vi "SDO_TRAJECTORY_EXECUTE_ABS.vi"(6 "EnableClosedLoop":bool=TRUE, 8 "Init":bool, 11 "End Pose ENG":T1={"TRANSLATION"={"X"=0.0, "Y"=0.0}, "ROTATION"={"VALUE"=0.0, "COS"=1.0, "SIN"=0.0}} {"ROTATION"."SIN" format="%13.4f"; "ROTATION"."COS" format="%13.4f"; "ROTATION"."VALUE" format="%13.4f"; "TRANSLATION"."Y" format="%14.3f"; "TRANSLATION"."X" format="%14.3f"}) -> (0 "AtReference":bool, 3 "Chassis Velocity Target":T4 {"vOmega" format="%10.3f"; "vY" format="%10.3f"; "vX" format="%10.3f"})   [LabVIEW 2019]
uses:
  <vilib>/Rock Robotics/WPI/ThirdParty/JAS_Junk/TrajLib/TypeDef/CHASSIS_SPEEDS.ctl
  <vilib>/Rock Robotics/WPI/ThirdParty/JAS_Junk/TrajLib/VI/Util_GetTime_U32.vi
  <vilib>/Rock Robotics/WPI/ThirdParty/JAS_Junk/TrajLib/ProfiledPIDController_NewPeriod.vi
  <vilib>/Rock Robotics/WPI/ThirdParty/JAS_Junk/TrajLib/ProfiledPIDController_SetIntegratorRange.vi
  <vilib>/Rock Robotics/WPI/ThirdParty/JAS_Junk/TrajLib/ProfiledPIDController_DisableContInput.vi
  <vilib>/Rock Robotics/WPI/ThirdParty/JAS_Junk/TrajLib/ProfiledPIDController_EnableContInput.vi
  <vilib>/Rock Robotics/WPI/ThirdParty/JAS_Junk/TrajLib/TrapProfConstraint_New.vi
  <vilib>/Rock Robotics/WPI/ThirdParty/JAS_Junk/TrajLib/Rotation2d_CreateAngle.vi
  <vilib>/Rock Robotics/WPI/ThirdParty/JAS_Junk/TrajLib/Translation2d_Create.vi
  <vilib>/Rock Robotics/WPI/ThirdParty/JAS_Junk/TrajLib/HolDrvCtrl_New.vi
  <vilib>/Rock Robotics/WPI/ThirdParty/JAS_Junk/TrajLib/HolDrvCtrl_PackPID.vi
  <vilib>/Rock Robotics/WPI/ThirdParty/JAS_Junk/TrajLib/HolDrvCtrl_SetTolerance.vi
  <vilib>/Rock Robotics/WPI/ThirdParty/JAS_Junk/TrajLib/HolDrvCtrl_SetEnabled.vi
  <vilib>/Rock Robotics/WPI/ThirdParty/JAS_Junk/TrajLib/HolDrvCtrl_Calculate_Trajectory.vi
  <vilib>/Rock Robotics/WPI/ThirdParty/JAS_Junk/TrajLib/HolDrvCtrl_AtReference.vi
  <vilib>/Rock Robotics/WPI/ThirdParty/JAS_Junk/TrajLib/TrapProfState_New.vi
  <vilib>/Rock Robotics/WPI/ThirdParty/JAS_Junk/TrajLib/PIDController_NewPeriod.vi
  <vilib>/Rock Robotics/SystemInterfaces/NetworkCommunication/NetComm_UsageReport_report.vi
  <vilib>/Rock Robotics/WPI/ThirdParty/JAS_Junk/TrajLib/PIDController_SetIntegratorRange.vi
  <vilib>/Rock Robotics/WPI/ThirdParty/JAS_Junk/TrajLib/PIDController_DisableContinousInput.vi
  <vilib>/Rock Robotics/WPI/ThirdParty/JAS_Junk/TrajLib/PIDController_EnableContinousInput.vi
  <vilib>/Rock Robotics/WPI/ThirdParty/JAS_Junk/TrajLib/Conv_Deg_Radians.vi
  <vilib>/Rock Robotics/WPI/ThirdParty/JAS_Junk/TrajLib/PIDController_Reset.vi
  <vilib>/Rock Robotics/WPI/ThirdParty/JAS_Junk/TrajLib/HolDrvCtrl_Calculate.vi
  <vilib>/Rock Robotics/WPI/ThirdParty/JAS_Junk/TrajLib/Rotation2d_GetRadians.vi
  <vilib>/Rock Robotics/WPI/ThirdParty/JAS_Junk/TrajLib/Rotation2d_GetAngleCosSin.vi
  <vilib>/Rock Robotics/WPI/ThirdParty/JAS_Junk/TrajLib/Pose2d_RelativeTo.vi
  <vilib>/Rock Robotics/WPI/ThirdParty/JAS_Junk/TrajLib/Pose2d_getRotation.vi
  <vilib>/Rock Robotics/WPI/ThirdParty/JAS_Junk/TrajLib/Rotation2d_Minus.vi
  <vilib>/Rock Robotics/WPI/ThirdParty/JAS_Junk/TrajLib/ProfiledPIDController_Calculate_Meas_Goal.vi
  <vilib>/Rock Robotics/WPI/ThirdParty/JAS_Junk/TrajLib/ChassisSpeeds_FromFieldRelativeSpeeds.vi
  <vilib>/Rock Robotics/WPI/ThirdParty/JAS_Junk/TrajLib/PIDController_Calculate_SP_PV.vi
  <vilib>/Rock Robotics/WPI/ThirdParty/JAS_Junk/TrajLib/ProfiledPIDController_Reset_PosOnly.vi
  <vilib>/Rock Robotics/WPI/ThirdParty/JAS_Junk/TrajLib/Rotation2d_Plus.vi
  <vilib>/Rock Robotics/WPI/ThirdParty/JAS_Junk/TrajLib/Transform2d_Create_PosePose.vi
  <vilib>/Rock Robotics/WPI/ThirdParty/JAS_Junk/TrajLib/Pose2d_New_TRRO.vi
  <vilib>/Rock Robotics/WPI/ThirdParty/JAS_Junk/TrajLib/Rotation2d_UnaryMinus.vi
  <vilib>/Rock Robotics/WPI/ThirdParty/JAS_Junk/TrajLib/Rotation2d_RotateBy.vi
  <vilib>/Rock Robotics/WPI/ThirdParty/JAS_Junk/TrajLib/ProfiledPIDController_SetGoal_PosOnly.vi
  <vilib>/Rock Robotics/WPI/ThirdParty/JAS_Junk/TrajLib/ProfiledPIDController_Calculate_Meas.vi
  <vilib>/Rock Robotics/WPI/ThirdParty/JAS_Junk/TrajLib/Rotation2d_GetCos.vi
  <vilib>/Rock Robotics/WPI/ThirdParty/JAS_Junk/TrajLib/Rotation2d_GetSin.vi
  <vilib>/Rock Robotics/WPI/ThirdParty/JAS_Junk/TrajLib/PIDController_SetSetpoint.vi
  <vilib>/Rock Robotics/WPI/ThirdParty/JAS_Junk/TrajLib/PIDController_Calculate_PV.vi
  <vilib>/Rock Robotics/WPI/ThirdParty/JAS_Junk/TrajLib/ProfiledPIDController_Reset.vi
  <vilib>/Rock Robotics/WPI/ThirdParty/JAS_Junk/TrajLib/Translation2d_RotateBy.vi
  <vilib>/Rock Robotics/WPI/ThirdParty/JAS_Junk/TrajLib/Translation2d_Minus.vi
  <vilib>/Rock Robotics/WPI/ThirdParty/JAS_Junk/TrajLib/Rotation2d_CreateXY.vi
  <vilib>/Rock Robotics/WPI/ThirdParty/JAS_Junk/TrajLib/ProfiledPIDController_SetGoal.vi
  <vilib>/Rock Robotics/WPI/ThirdParty/JAS_Junk/TrajLib/TrapProfile_New.vi
  <vilib>/Rock Robotics/WPI/ThirdParty/JAS_Junk/TrajLib/ProfiledPIDController_GetPeriod.vi
  <vilib>/Rock Robotics/WPI/ThirdParty/JAS_Junk/TrajLib/TrapProfile_Calculate.vi
  <vilib>/Rock Robotics/WPI/ThirdParty/JAS_Junk/TrajLib/ControllerUtil_GetModulusError.vi
  <vilib>/Rock Robotics/WPI/ThirdParty/JAS_Junk/TrajLib/Util_CalcDist.vi
  <vilib>/Rock Robotics/WPI/ThirdParty/JAS_Junk/TrajLib/TrapProfile_ShouldFlipAcceleration.vi
  <vilib>/Rock Robotics/WPI/ThirdParty/JAS_Junk/TrajLib/TrapProfile_Direct.vi
  <vilib>/Rock Robotics/WPI/ThirdParty/JAS_Junk/TrajLib/PIDController_GetPeriod.vi
  Swerve_Drive_System/SDO_DRIVE_GLOBALS.vi
  <vilib>/Rock Robotics/WPI/ThirdParty/JAS_Junk/TrajLib/VI/Util_GetTime_U64.vi
  SDO_TRAJECTORY_GLOBALS.vi
  <vilib>/Rock Robotics/WPI/ThirdParty/JAS_Junk/TrajLib/Globals/Util_LibraryGlobals.vi
  <vilib>/Rock Robotics/WPI/ThirdParty/JAS_Junk/TrajLib/Trajectory_Library.lvlib
  <vilib>/Rock Robotics/WPI/ThirdParty/JAS_Junk/TrajLib/TypeDef/TRANSLATION2D.ctl
  <vilib>/Rock Robotics/WPI/ThirdParty/JAS_Junk/TrajLib/TypeDef/ROTATION2D.ctl
  <vilib>/Rock Robotics/WPI/ThirdParty/JAS_Junk/TrajLib/TypeDef/POSE2D.ctl
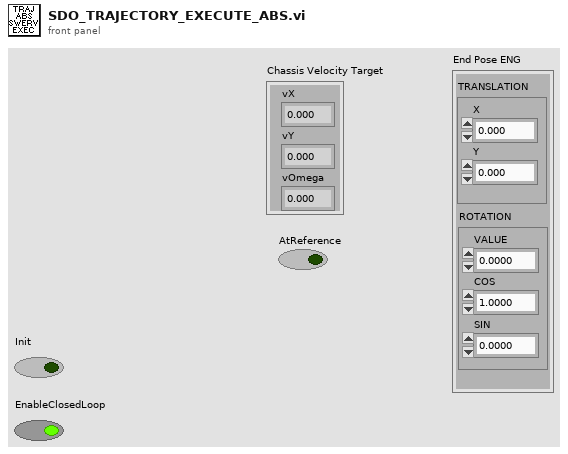
[diagram p1: front panel]
types:
  T1 = typedef "Trajectory_Library.lvlib/POSE2D.ctl" = cluster{"TRANSLATION":T2, "ROTATION":T3}
  T2 = typedef "Trajectory_Library.lvlib/TRANSLATION2D.ctl" = cluster{"X":dbl, "Y":dbl}
  T3 = typedef "Trajectory_Library.lvlib/ROTATION2D.ctl" = cluster{"VALUE":dbl, "COS":dbl, "SIN":dbl}
  T4 = typedef "Trajectory_Library.lvlib/CHASSIS_SPEEDS.ctl" = cluster{"vX":dbl, "vY":dbl, "vOmega":dbl}
  T5 = typedef "Trajectory_Library.lvlib/SWERVE_DRIVE_KINEMATICS.ctl" = cluster{"NumModules":i32, "InverseKinematics":T6, "ForwardKinematics":T6, "Modules":T2[], "PrevCoR":T2, "SavedModuleStates":T7[]}
  T6 = typedef "NI_Matrix.lvlib/RealMatrix.ctl" = dbl[][]
  T7 = typedef "Trajectory_Library.lvlib/SWERVE_DRIVE_MODULE_STATE.ctl" = cluster{"Speed":dbl, "Angle":T3}
  T8 = typedef "Trajectory_Library.lvlib/TRAJECTORY.ctl" = cluster{"TotalTImeSecs":dbl, "States":T9[]}
  T9 = typedef "Trajectory_Library.lvlib/TRAJ_STATE.ctl" = cluster{"TimeSeconds":dbl, "Velocity":dbl, "Acceleration":dbl, "POSE":T1, "Curvature":dbl}
  T10 = typedef "Trajectory_Library.lvlib/PID_TUNING.ctl" = cluster{"Kp":dbl, "Ki":dbl, "Kd":dbl, "MaximumIntegral":dbl, "MinimumIntegral":dbl}
  T11 = typedef "Trajectory_Library.lvlib/PROFILED_PID_CONTROLLER.ctl" = cluster{"Controller":T12, "Goal":T13, "Setpoint":T13, "Constraint":T14}
  T12 = typedef "Trajectory_Library.lvlib/PID_CONTROLLER.ctl" = cluster{"Kp":dbl, "Ki":dbl, "Kd":dbl, "Period":dbl, "Max_Integral":dbl, "Min_Integral":dbl, "Max_Input":dbl, "Min_Input":dbl, "Continuous":bool, "PositionError":dbl, "VelocityError":dbl, "PrevError":dbl, "TotalError":dbl, "PositionTolerance":dbl, "VelocityTolerance":dbl, "SetPoint":dbl, "Kf":dbl, "Prev_Deriv":dbl, "Prev_Deriv 2":dbl, "DerivativeFilter":bool, "Min_Output":dbl, "Max_Output":dbl, "Prev_F_P":dbl, "Prev_F_P_2":dbl, "AntiWindupActive":bool, "Measurement":dbl}
  T13 = typedef "Trajectory_Library.lvlib/TRAPEZOID_PROFILE_STATE.ctl" = cluster{"Position":dbl, "Velocity":dbl}
  T14 = typedef "Trajectory_Library.lvlib/TRAPEZOID_PROFILE_CONSTRAINT.ctl" = cluster{"MaxVelocity":dbl, "MaxAcceleration":dbl}
  T15 = typedef "Trajectory_Library.lvlib/HOLONOMIC_PACK_TUNING.ctl" = cluster{"X PID Tuning":T10, "Y PID Tuning":T10, "thetaProfiledPID_CTRL":T11}
  T16 = typedef "Trajectory_Library.lvlib/HOLONOMIC_DRV_CTRL.ctl" = cluster{"poseTolerance":T1, "poseError":T1, "Enabled":bool, "PID_xCtrl":T12, "PID_yCtrl":T12, "PROF_PID_thetaCtrl":T11, "RotationError":T3, "FirstRun":bool}
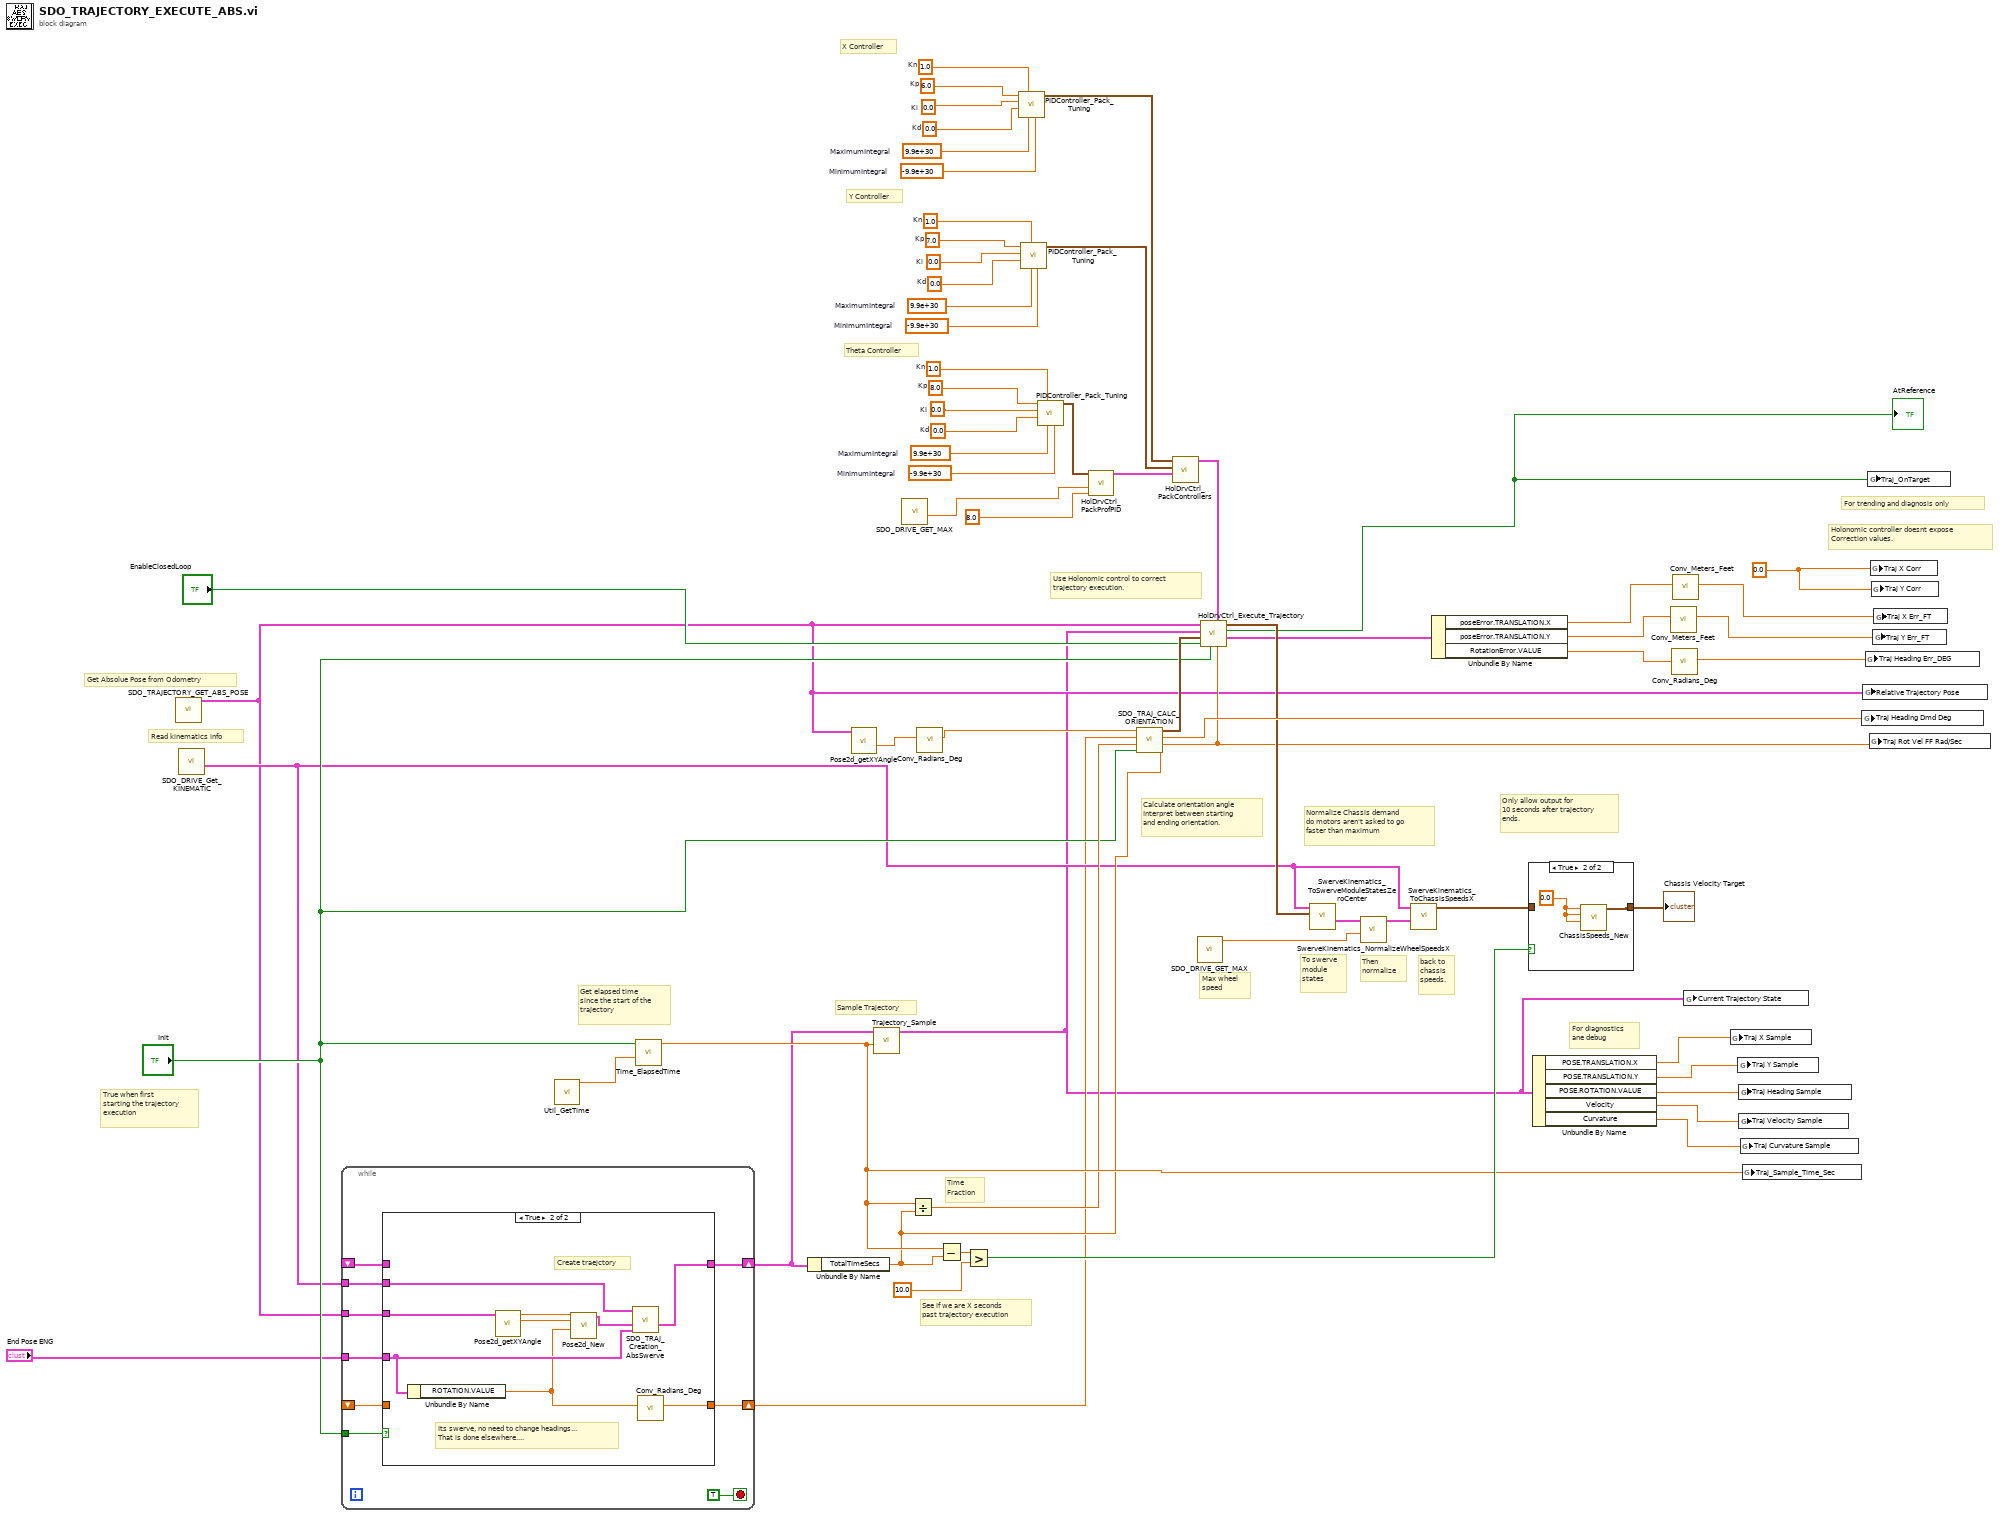
[diagram p0: block diagram]
diagram:
  w23 = 1.0  # Kn
  w26 = 8.0  # Kp
  w35 = 0.0  # Ki
  w36 = 0.0  # Kd
  w37 = 9.9e+30  # MaximumIntegral
  w38 = -9.9e+30  # MinimumIntegral
  w21 = 1.0  # Kn
  w24 = 6.0  # Kp
  w27 = 0.0  # Ki
  w28 = 0.0  # Kd
  w29 = 9.9e+30  # MaximumIntegral
  w30 = -9.9e+30  # MinimumIntegral
  w22 = 1.0  # Kn
  w25 = 7.0  # Kp
  w31 = 0.0  # Ki
  w32 = 0.0  # Kd
  w33 = 9.9e+30  # MaximumIntegral
  w34 = -9.9e+30  # MinimumIntegral
  w51 = 0.0 ("Y Corr")
  # "Theta Controller"
  # "Y Controller"
  # "X Controller"
  # "Time\nFraction"
  # "Calculate orientation angle\nInterpret between starting\nand ending orientation."
  # "Max wheel\nspeed"
  # "True when first\nstarting the trajectory\nexecution"
  # "Get elapsed time\nsince the start of the\ntrajectory"
  # "Holonomic controller doesnt expose\nCorrection values."
  # "Normalize Chassis demand\ndo motors aren't asked to go\nfaster than maximum"
  # "Use Holonomic control to correct\ntrajectory execution."
  # "For trending and diagnosis only"
  # "For diagnostics\nane debug"
  # "Get Absolue Pose from Odometry"
  # "back to\nchassis\nspeeds."
  # "Then\nnormalize"
  # "To swerve\nmodule\nstates"
  # "Read kinematics info"
  # "Sample Trajectory"
  # "See if we are X seconds \npast trajectory execution"
  # "Only allow output for\n10 seconds after trajectory\nends."
  n1 = call "SDO_TRAJECTORY_GET_ABS_POSE.vi"() -> ("Absolute Odometry Pose"=w6:T1)  [unwired: 11 in]
  n2 = call "SDO_DRIVE_Get_KINEMATIC.vi"() -> ("out SWERVE_DRIVE_KINEMATICS"=w8:T5)  [unwired: 11 in]
  n3 = while {
    tunnel: "Init" -> [w73]
    tunnel: w8 -> [w72]
    tunnel: w6 -> [w71]
    shift-right: [w70] -> w7
    shift-left: _ -> [w69]
    shift-right: [w68] -> w3
    shift-left: _ -> [w67]
    tunnel: "End Pose ENG" -> [w66]
    stop <- TRUE stop-if-true
    n4 = case shown="True" w73 {
      tunnel: w72 -> [_ w85]
      tunnel: w71 -> [_ w83]
      tunnel: [w76 w84] -> w70
      tunnel: w69 -> [w76 _]
      tunnel: [w75 w78] -> w68
      tunnel: w67 -> [w75 _]
      tunnel: w66 -> [_ w79]
      frame False {
      }
      frame True {
        # "Its swerve, no need to change headings...\nThat is done elsewhere...."
        # "Create traejctory"
        n5 = Unbundle By Name(w79) -> ("ROTATION.VALUE"=w77:dbl)
        n6 = call <vilib>:"Pose2d_getXYAngle.vi"("in POSE"=w83) -> ("Y"=w81:dbl, "X"=w82:dbl)  [unwired: 8 in, 1 out]
        n7 = call <vilib>:"Pose2d_New.vi"("Heading"=w77, "Y"=w81, "X"=w82) -> ("out POSe"=w80:T1)  [unwired: 8 in]
        n8 = call "SDO_TRAJ_Creation_AbsSwerve.vi"("End Pose  ENG"=w79, "Current Pose SI"=w80, "SWERVE_DRIVE_KINEMATICS"=w85) -> ("Absolute Trajectory"=w84:T8)  [unwired: 6 in, 2 out]
        n9 = call <vilib>:"Conv_Radians_Deg.vi"("Radians"=w77) -> ("Degrees"=w78:dbl)  [unwired: 10 in]
      }
    }
  }
  n10 = call <vilib>:"Util_GetTime.vi"() -> ("FPGA_Time_Seconds"=w57:dbl)  [unwired: 9 in, 2 out]
  n11 = call <vilib>:"Time_ElapsedTime.vi"("PassthroughTime_SEC"=w57, "Reset"="Init") -> ("Elapsed Time Sec"=w49:dbl)  [unwired: 9 in]
  n12 = Unbundle By Name(w7) -> ("TotalTImeSecs"=w12:dbl)
  n13 = call <vilib>:"Pose2d_getXYAngle.vi"("in POSE"=w6) -> ("Angle"=w5:dbl)  [unwired: 8 in, 2 out]
  n14 = call <vilib>:"Trajectory_Sample.vi"("Time"=w49, "InputTRAJECTORY"=w7) -> ("OutputTRAJ_STATE"=w2:T9)  [unwired: 9 in]
  n15 = call "SDO_DRIVE_GET_MAX.vi"() -> ("Max Rotational Vel (Rad/Sec)"=w11:dbl)  [unwired: 10 in, 1 out]
  n16 = Divide(x=w49, y=w12) -> (x/y=w48:dbl)
  n17 = call <vilib>:"Conv_Radians_Deg.vi"("Radians"=w5) -> ("Degrees"=w4:dbl)  [unwired: 10 in]
  n18 = Subtract(x=w49, y=w12) -> (x-y=w65:dbl)
  n19 = Greater?(x=w65, y=10.0) -> (0:w63:bool)
  n20 = call <vilib>:"PIDController_Pack_Tuning.vi"("MinimumIntegral"=w30, "MaximumIntegral"=w29, "Kn"=w21, "Kd"=w28, "Ki"=w27, "Kp"=w24) -> ("PID Tuning"=w39:T10)  [unwired: 5 in]
  n21 = call <vilib>:"PIDController_Pack_Tuning.vi"("MinimumIntegral"=w34, "MaximumIntegral"=w33, "Kn"=w22, "Kd"=w32, "Ki"=w31, "Kp"=w25) -> ("PID Tuning"=w40:T10)  [unwired: 5 in]
  n22 = call <vilib>:"PIDController_Pack_Tuning.vi"("MinimumIntegral"=w38, "MaximumIntegral"=w37, "Kn"=w23, "Kd"=w36, "Ki"=w35, "Kp"=w26) -> ("PID Tuning"=w20:T10)  [unwired: 5 in]
  n23 = call <vilib>:"HolDrvCtrl_PackProfPID.vi"("Max Accel"=8.0, "Max Speed"=w11, "Theta PID Tuning"=w20) -> ("Theta PID CONTROLLER"=w41:T11)  [unwired: 8 in]
  n24 = call "SDO_TRAJ_CALC_ORIENTATION.vi"("Total Trajectory Time"=w12, "Init"="Init", "Time Fraction"=w48, "End Orientation Demand DEG"=w3, "Starting Orientation  DEG"=w4) -> ("Rotational Velocity"=w15:dbl, "Orientation Demand Deg"=w50:dbl, "Orientation Demand"=w19:T3)  [unwired: 4 in]
  n25 = call <vilib>:"HolDrvCtrl_PackControllers.vi"("thetaProfiledPID_CTRL"=w41, "Y PID Tuning"=w40, "X PID Tuning"=w39) -> ("HOLONOMIC_CTRL_PACK_TUNING"=w42:T15)  [unwired: 8 in]
  n26 = call "SDO_DRIVE_GET_MAX.vi"() -> ("Max Wheel Vel (Meter/Sec)"=w59:dbl)  [unwired: 10 in, 1 out]
  n27 = call <vilib>:"HolDrvCtrl_Execute_Trajectory.vi"("Rotational Velocity Feedforward \nRad/Sec"=w15, "HOLONOMIC_CTRL_PACK_TUNING"=w42, "Reset"="Init", "Enable"="EnableClosedLoop", "angleRef"=w19, "desiredTrajState"=w2, "currentPose"=w6) -> ("outHOLONOMIC_DRV_CTRL"=w16:T16, "AtReference"=w17:bool, "calcChassisSpeed"=w18:T4)  [unwired: 2 in]
  "AtReference" <- w17
  n28 = call <vilib>:"SwerveKinematics_ToSwerveModuleStatesZeroCenter.vi"("ChassisSpeeds"=w18, "in SWERVE_DRIVE_KINEMATICS"=w8) -> ("ModuleStates"=w62:T7[])  [unwired: 8 in, 1 out]
  n29 = call <vilib>:"SwerveKinematics_NormalizeWheelSpeedsX.vi"("AttainableMaxSpeed"=w59, "in WheelStates"=w62) -> ("out WheelStates"=w61:T7[])  [unwired: 9 in]
  n30 = call <vilib>:"SwerveKinematics_ToChassisSpeedsX.vi"("WheelStates"=w61, "in SWERVE_DRIVE_KINEMATICS"=w8) -> ("Chassis Speed"=w58:T4)  [unwired: 9 in]
  n31 = Unbundle By Name(w16) -> ("poseError.TRANSLATION.X"=w46:dbl, "poseError.TRANSLATION.Y"=w45:dbl, "RotationError.VALUE"=w13:dbl)
  n32 = case shown="True" w63 {
    tunnel: w58 -> [w86 _]
    tunnel: [w86 w87] -> w60
    frame False {
    }
    frame True {
      w88 = 0.0 ("vX")
      n33 = call <vilib>:"ChassisSpeeds_New.vi"("vAngular"=w88, "vY"=w88, "vX"=w88) -> ("CHASSIS"=w87:T4)  [unwired: 8 in]
    }
  }
  "Chassis Velocity Target" <- w60
  n34 = Unbundle By Name(w2) -> ("POSE.TRANSLATION.X"=w56:dbl, "POSE.TRANSLATION.Y"=w55:dbl, "POSE.ROTATION.VALUE"=w54:dbl, "Velocity"=w53:dbl, "Curvature"=w52:dbl)
  n35 = call <vilib>:"Conv_Meters_Feet.vi"("Meters"=w45) -> ("Feet"=w44:dbl)  [unwired: 10 in]
  n36 = call <vilib>:"Conv_Radians_Deg.vi"("Radians"=w13) -> ("Degrees"=w47:dbl)  [unwired: 10 in]
  n37 = call <vilib>:"Conv_Meters_Feet.vi"("Meters"=w46) -> ("Feet"=w43:dbl)  [unwired: 10 in]
  n38 = global write "SDO_TRAJECTORY_GLOBALS.vi" "Current Trajectory State"(w2) -> ()
  n39 = global write "SDO_TRAJECTORY_GLOBALS.vi" "Traj X Sample"(w56) -> ()
  n40 = global write "SDO_TRAJECTORY_GLOBALS.vi" "Traj Y Sample"(w55) -> ()
  n41 = global write "SDO_TRAJECTORY_GLOBALS.vi" "Traj Heading Sample"(w54) -> ()
  n42 = global write "SDO_TRAJECTORY_GLOBALS.vi" "Traj Velocity Sample"(w53) -> ()
  n43 = global write "SDO_TRAJECTORY_GLOBALS.vi" "Traj Curvature Sample"(w52) -> ()
  n44 = global write "SDO_TRAJECTORY_GLOBALS.vi" "Traj_Sample_Time_Sec"(w49) -> ()
  n45 = global write "SDO_TRAJECTORY_GLOBALS.vi" "Traj Heading Dmd Deg"(w50) -> ()
  n46 = global write "SDO_TRAJECTORY_GLOBALS.vi" "Relative Trajectory Pose"(w6) -> ()
  n47 = global write "SDO_TRAJECTORY_GLOBALS.vi" "Traj Heading Err_DEG"(w47) -> ()
  n48 = global write "SDO_TRAJECTORY_GLOBALS.vi" "Traj_OnTarget"(w17) -> ()
  n49 = global write "SDO_TRAJECTORY_GLOBALS.vi" "Traj Rot Vel FF Rad/Sec"(w15) -> ()
  n50 = global write "SDO_TRAJECTORY_GLOBALS.vi" "Traj X Corr"(w51) -> ()
  n51 = global write "SDO_TRAJECTORY_GLOBALS.vi" "Traj Y Corr"(w51) -> ()
  n52 = global write "SDO_TRAJECTORY_GLOBALS.vi" "Traj Y Err_FT"(w44) -> ()
  n53 = global write "SDO_TRAJECTORY_GLOBALS.vi" "Traj X Err_FT"(w43) -> ()
